vi "Get Queues.vi"(8 "error in (no error)":errorcluster, 11 "MCP SSE Response in":refnum<class "MCP SSE Response.lvclass">) -> (0 "error out":errorcluster, 1 "cancelled":refnum<queue>, 2 "events":refnum<queue>, 3 "MCP SSE Response out":refnum<class "MCP SSE Response.lvclass">)   [LabVIEW 2020, in "MCP Server.lvlib" / "MCP SSE Response.lvclass"]
doc: "Returns the two queues held by an MCP SSE Response: the events queue (one complete, formatted SSE event text per element; an empty string ends the stream) and the single-element cancelled flag queue, which holds TRUE once the client has gone away."
uses:
  MCP SSE Response.lvclass
  MCP SSE Response.lvclass/MCP SSE Response.ctl
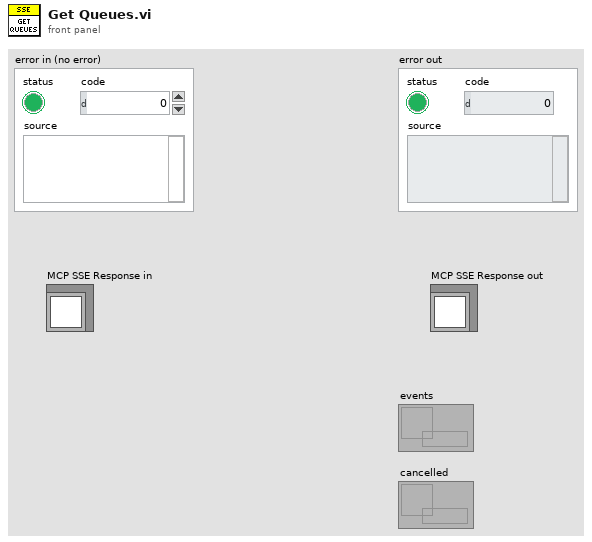
[diagram p1: front panel]
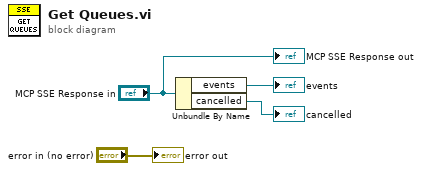
[diagram p0: block diagram]
diagram:
  n1 = Unbundle By Name("MCP SSE Response in") -> ("events"=→"events":refnum<queue>, "cancelled"=→"cancelled":refnum<queue>)
  "error out" <- "error in (no error)"
  "MCP SSE Response out" <- "MCP SSE Response in"
